vi "Sets the Date and Time.vi"(5 "Enable to Query":bool=TRUE, 7 "Enable to Sets":bool, 8 "error in":errorcluster, 10 "Date and Time":timestamp=timestamp(3029529600 s since 1904-01-01) format="%<%Y/%m/%d\n%H:%M:%S>T", 11 "VISA resource name":refnum<visa-resource-name>) -> (0 "error out":errorcluster, 1 "Time":string, 2 "Date":string, 3 "VISA resource name out":refnum<visa-resource-name>)   [LabVIEW 2012, in "GDM-9052.lvlib"]
uses:
  GDM-9052.lvlib
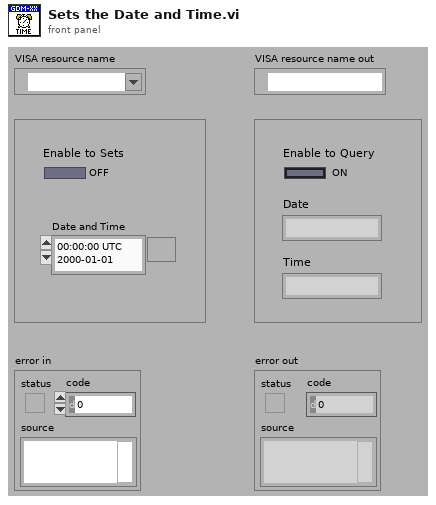
[diagram p1: front panel]
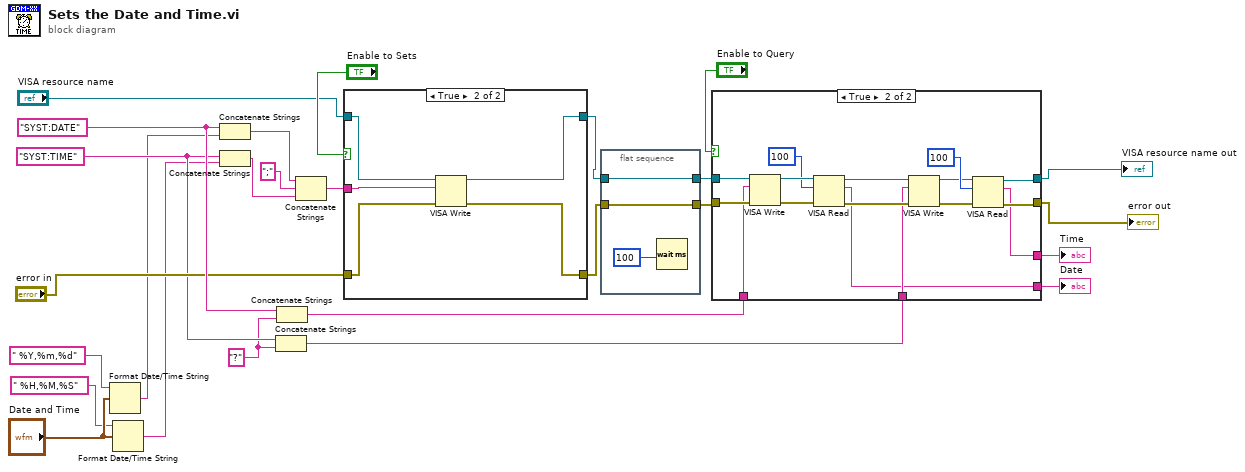
[diagram p0: block diagram]
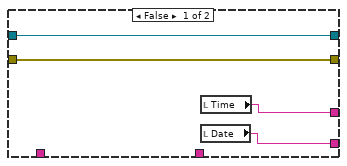
[diagram p2: hidden frame]
diagram:
  w18 = "SYST:TIME"
  w16 = "?"
  w26 = "SYST:DATE"
  n1 = Format Date/Time String(time format string (%c)=" %Y,%m,%d", seconds (now)="Date and Time") -> (date/time string=w6:string)  [unwired: 1 in]
  n2 = Format Date/Time String(time format string (%c)=" %H,%M,%S", seconds (now)="Date and Time") -> (date/time string=w5:string)  [unwired: 1 in]
  n3 = Concatenate Strings(w26, w6) -> (w15:string)
  n4 = Concatenate Strings(w18, w5) -> (w14:string)
  n5 = Concatenate Strings(w18, w16) -> (w17:string)
  n6 = Concatenate Strings(w26, w16) -> (w21:string)
  n7 = Concatenate Strings(w15, ";" ("string"), w14) -> (w12:string)
  n8 = case shown="True" "Enable to Sets" {
    tunnel: "VISA resource name" -> [w28 w33]
    tunnel: "error in" -> [w27 w32]
    tunnel: [w28 w31] -> w4
    tunnel: [w27 w30] -> w2
    tunnel: w12 -> [_ w29]
    frame False {
    }
    frame True {
      n9 = VISA Write(VISA resource name=w33, write buffer=w29, error in (no error)=w32) -> (VISA resource name out=w31:refnum<visa-resource-name>, error out=w30:errorcluster)  [unwired: 1 out]
    }
  }
  n10 = flat-sequence {
    tunnel: w4 -> [w36]
    tunnel: [w36] -> w3
    tunnel: w2 -> [w35]
    tunnel: [w35] -> w1
    frame #0 {
      n11 = Wait (ms)(milliseconds to wait=u32 100) -> ()  [unwired: 1 out]
    }
  }
  n12 = case shown="True" "Enable to Query" {
    tunnel: w3 -> [w40 w56]
    tunnel: w1 -> [w39 w55]
    tunnel: w21 -> [_ w54]
    tunnel: [w40 w45] -> w20
    tunnel: [w39 w44] -> w19
    tunnel: w17 -> [_ w43]
    tunnel: [w38 w42] -> w11
    tunnel: [w37 w41] -> w10
    frame False {
      n13 = local read "Time"() -> (w38:string)
      n14 = local read "Date"() -> (w37:string)
    }
    frame True {
      n15 = VISA Write(VISA resource name=w56, write buffer=w54, error in (no error)=w55) -> (VISA resource name out=w53:refnum<visa-resource-name>, error out=w52:errorcluster)  [unwired: 1 out]
      n16 = VISA Read(VISA resource name=w53, byte count=u32 100, error in (no error)=w52) -> (VISA resource name out=w47:refnum<visa-resource-name>, read buffer=w41:string, error out=w46:errorcluster)  [unwired: 1 out]
      n17 = VISA Write(VISA resource name=w47, write buffer=w43, error in (no error)=w46) -> (VISA resource name out=w48:refnum<visa-resource-name>, error out=w49:errorcluster)  [unwired: 1 out]
      n18 = VISA Read(VISA resource name=w48, byte count=u32 100, error in (no error)=w49) -> (VISA resource name out=w45:refnum<visa-resource-name>, read buffer=w42:string, error out=w44:errorcluster)  [unwired: 1 out]
    }
  }
  "VISA resource name out" <- w20
  "error out" <- w19
  "Time" <- w11
  "Date" <- w10
